vi "MQTT QoS - Confirm Reception.vi"(0 "MQTT Reference":T2, 5 "PacketID":u16, 7 "MessageType":T1=enum."PUBREC", 11 "Error In":errorcluster) -> (4 "MQTT Reference":T2, 6 "Released Message":u8[](array[numeric]), 8 "Found?":bool, 15 "Error Out":errorcluster)   [LabVIEW 2019, in "KoRE-MQTT.lvlib"]
doc: "Copyright (c) 2025 KoRElibs.com\nSPDX-License-Identifier: EUPL-1.2\n\nThis VI is licensed under the European Union Public License (EUPL) Version 1.2. You may use this VI unmodified in proprietary works. If you distribute a modified version of this file, the modified file must be released under the EUPL-1.2. Full license: https://joinup.ec.europa.eu/asset/eupl/eupl/1.2/"
uses:
  KoRE-MQTT.lvlib
  Public/TypeDefs/MQTT Client Session.ctl
  TypeDefs/MQTT Packet - Type.ctl
  TypeDefs/MQTT Client Session - Data Value Reference.ctl
  Public/TypeDefs/MQTT Client Session - Data.ctl
  Public/TypeDefs/MQTT Property - Will.ctl
  Public/TypeDefs/MQTT Property - CONNECT.ctl
  TypeDefs/MQTT Subscription - Info.ctl
  TypeDefs/MQTT QoS - In-flight Data.ctl
panel:
  out "Debug Info":variant
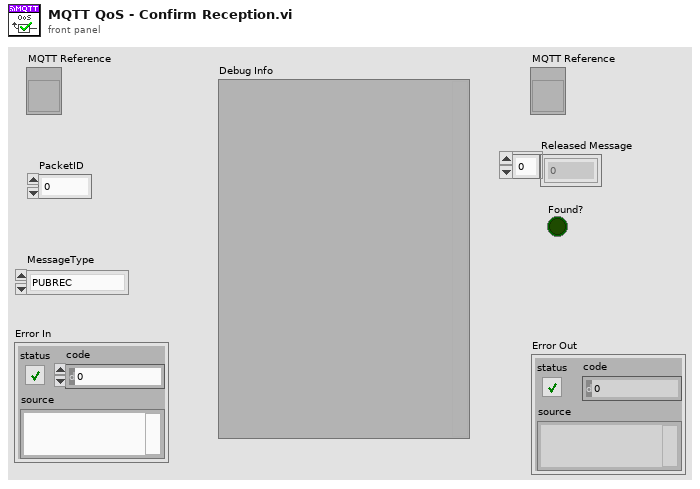
[diagram p1: front panel]
types:
  T1 = typedef "KoRE-MQTT.lvlib/MQTT Packet - Type.ctl" = enum32{"Reserved", "CONNECT", "CONNACK", "PUBLISH", "PUBACK", "PUBREC", "PUBREL", "PUBCOMP", "SUBSCRIBE", "SUBACK", "UNSUBSCRIBE", "UNSUBACK", "PINGREQ", "PINGRESP", "DISCONNECT", "AUTH"}
  T2 = typedef "KoRE-MQTT.lvlib/MQTT Client Session.ctl" = refnum<vi>
  T3 = typedef "KoRE-MQTT.lvlib/MQTT Client Session - Data Value Reference.ctl" = refnum<data-value>
  T4 = typedef "KoRE-MQTT.lvlib/MQTT QoS - In-flight Data.ctl" = cluster{"Time":u32, "Message":u8[]}
  T5 = typedef "KoRE-MQTT.lvlib/MQTT Client Session - Data.ctl" = cluster{"TCP ref":refnum<k5>, "Next Packet Id":u16, "Version":u8, "Host":string, "Port":u16, "Ping Delta":u32, "Username":string, "Password":string, "Will QoS":u8, "Will Retain":bool, "Will Topic":string, "Will Payload":string, "TCP Timeout":i32, "Semaphore":T6, "In-Flight Messages":variant, "Close":bool, "Last Send":u32, "Keep Alive":u16, "Last Ping RTT":u32, "Last Ping":u32, "Will Properties":T7[], "Session Expiry Interval":u32, "Maximum QoS":u8, "Retain Available":bool, "Server Maximum Packet Size":u32, "Client Identifier":string, "Server Topic Alias Maximum":u16, "Wildcard Subscription Available":bool, "Subscription Identifier Available":bool, "Shared Subscription Available":bool, "Connect Properties":T8[], "Client Maximum Packet Size":u32, "Client Topic Alias Maximum":u16, "Server Receive Maximum":u16, "Client Receive Maximum":u16, "TLS cfg":refnum<k36>, "Subscriptions":T9[]}
  T6 = typedef "Semaphore RefNum" = refnum<k1>
  T7 = typedef "KoRE-MQTT.lvlib/MQTT Property - Will.ctl" = cluster{"Property":u8, "Value":string}
  T8 = typedef "KoRE-MQTT.lvlib/MQTT Property - CONNECT.ctl" = cluster{"Property":u8, "Value":string}
  T9 = typedef "KoRE-MQTT.lvlib/MQTT Subscription - Info.ctl" = cluster{"Packet Id":u16, "Index":u16, "Identifier":u32, "QoS":u8, "Topic Filter":string, "Reason Code":u8, "Reason String":string, "Granted":bool}
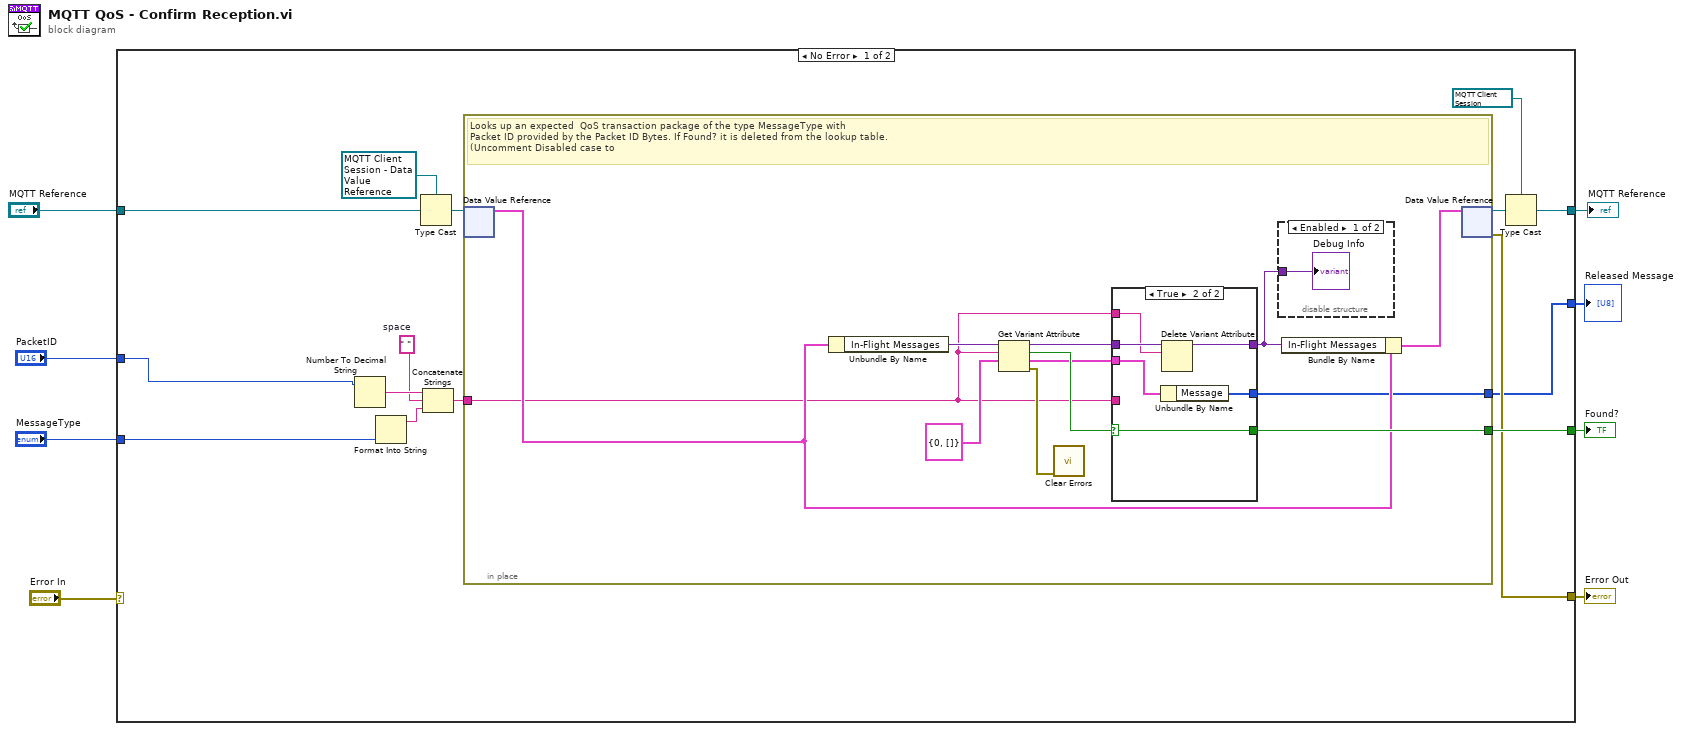
[diagram p0: block diagram]
diagram:
  n1 = case shown="No Error" "Error In" {
    tunnel: [w19 w45] -> w8
    tunnel: [w13 _] -> w7
    tunnel: [w18 _] -> w6
    tunnel: "PacketID" -> [w10 _]
    tunnel: "MessageType" -> [w14 _]
    tunnel: "MQTT Reference" -> [w12 w45]
    tunnel: [w9 _] -> w1
    frame No Error {
      w11 = " "  # space
      n2 = Number To Decimal String(number=w10) -> (decimal integer string=w17:string)  [unwired: 1 in]
      n3 = Format Into String(w14) -> (resulting string=w16:string)  [unwired: 3 in, 1 out]
      n4 = Type Cast(type=T3 refnum ("data value reference"), x=w12) -> (*(type *) &x=w23:T3)
      n5 = Concatenate Strings(w17, w11, w16) -> (w15:string)
      n6 = in-place {
        in-place-border: [w30] -> w18
        in-place-border: w15 -> [w24]
        in-place-border: [w25] -> w9
        # "Looks up an expected  QoS transaction package of the type MessageType with \nPacket ID provided by the Packet ID Bytes. If Found? it is deleted from the lookup table.\n(Uncomment Disabled case to"
        n7 = in-place-dvr #1(w23) -> (w29:T5)  [unwired: 1 out]
        n8 = Unbundle By Name(w29) -> ("In-Flight Messages"=w34:variant)
        n9 = Get Variant Attribute(Variant=w34, name=w24, default value (empty Variant)=T4 {"Time"=0, "Message"=[]}) -> (duplicate Variant=w33:variant, found=w27:bool, value=w26:T4, error out=w32:errorcluster)  [unwired: 1 in]
        n10 = call <vilib>:"Clear Errors.vi"("error in (no error)"=w32) -> ()  [unwired: 5 in, 2 out]
        n11 = case shown="True" w27 {
          selector: w27 -> [w37 w42]
          tunnel: w33 -> [w38 w44]
          tunnel: [w38 w43] -> w31
          tunnel: [w37 w42] -> w30
          tunnel: w24 -> [_ _]
          tunnel: w26 -> [_ w41]
          tunnel: [_ w40] -> w25
          tunnel: w24 -> [_ w39]
          frame False {
            # "#todo: handle unexpected response package (not expected in-flight)"
          }
          frame True {
            n12 = Unbundle By Name(w41) -> ("Message"=w40:u8[])
            n13 = Delete Variant Attribute(6:w39, 7:w44) -> (3:w43:variant)  [unwired: 1 in, 2 out]
          }
        }
        n14 = disable-structure shown="Enabled" {
          disable-tunnel: w31 -> [w36 _]
          frame Enabled {
            "Debug Info" <- w36
          }
          frame Disabled {
          }
        }
        n15 = Bundle By Name(cluster=w29, "In-Flight Messages"=w31) -> (w35:T5)
        n16 = in-place-dvr #1(w35) -> (w21:T3, w13:errorcluster)
      }
      n17 = Type Cast(type=T2 refnum ("mqtt ref"), x=w21) -> (*(type *) &x=w19:T2)
    }
    frame Error {
    }
  }
  "MQTT Reference" <- w8
  "Error Out" <- w7
  "Found?" <- w6
  "Released Message" <- w1
